vi "eDyno NVH Accel + RPM Simulator.vi"() -> ()   [LabVIEW 2026]
doc: "eDyno NVH simulator for ORDER ANALYSIS - PXIe-4468 AO0 + AO1 in ONE task (the 4468 AO channels share one timing engine, so they cannot run as two separate tasks).\n\nAO0 = accelerometer: PCB 356A15 (one axis) at Sensitivity mV/g, with the same speed profile and Fault Injection as eDyno NVH Accel Simulator.vi.\nAO1 = motor-shaft speed reference, phase-locked to AO0 (same shaft phase, same samples):\n- Pulse Tach OFF (default): analog voltage proportional to rpm, Tach Scale V per 1000 rpm (default 1 V/1000 rpm, so 4500 rpm = 4.5 V).\n- Pulse Tach ON: once-per-rev square wave, 0 / Pulse High V (default 5 V), 50 % duty, rising edge at shaft angle 0 - a keyphasor for SVT tach-to-speed conversion (1 pulse/rev).\n\nAcquire in a separate VI: AO0 -> an accel AI channel (IEPE OFF, same mV/g), AO1 -> a voltage AI channel (IEPE OFF), both in one AI task so they share the sample clock. Analog mode: rpm = V x 1000 / Tach Scale. Orders are referred to the MOTOR shaft (1x = rpm/60 Hz). Fault Frequencies is the answer key at the current speed.\n\nDefaults: run-up 500 -> 4500 rpm over 30 s (Speed Profile / Run-up Enabled), or constant 3000 rpm. Timing: 3-block AO buffer, DAQmx Write paces the loop, the first write auto-starts the task."
uses:
  <vilib>/DAQmx/miscellaneous.llb/DAQmx Fill In Error Info.vi
panel:
  out "Tach Output (V)":dbl[](graph)
  out "Simulated Acceleration (g)":dbl[](graph)
  out "Fault Frequencies (Hz)":T1={"1x Shaft"=50.0, "2x Misalign"=100.0, "BPFO"=178.5, "Torque Ripple"=1200.0, "PWM Carrier"=16000.0}
  out "Shaft Speed (rpm)":dbl=3000.0
  in  "STOP":bool
  in  "Tach Output":T2={"Pulse Tach 1ppr (OFF = analog rpm)"=FALSE, "Tach Scale (V per 1000 rpm)"=1.0, "Pulse High (V)"=5.0}
  in  "Speed Profile":T3={"Run-up Enabled"=FALSE, "Constant Speed (rpm)"=3000.0, "Run-up Start (rpm)"=500.0, "Run-up End (rpm)"=4500.0, "Run-up Duration (s)"=30.0}
  in  "Sim Config":T4={"Sample Rate (Hz)"=51200.0, "Ref Speed (rpm)"=3000.0, "Baseline 1x (g)"=0.02, "Noise Floor (g rms)"=0.01, "BPFO Order"=3.57, "Resonance (Hz)"=3500.0, "Decay (ms)"=0.8, "Pole Pairs"=4.0, "PWM Carrier (Hz)"=16000.0}
  in  "Fault Injection":T5={"Imbalance ON"=FALSE, "Imbalance (g)"=0.5, "Misalignment ON"=FALSE, "Misalignment (g)"=0.2, "Bearing BPFO ON"=FALSE, "Bearing Impact (g)"=2.0, "Motor Ripple ON"=FALSE, "Torque Ripple (g)"=0.3, "PWM Noise ON"=FALSE, "PWM Level (g)"=0.05}
  in  "DAQ Settings":T6={"Device"="PXI2Slot4", "AO Channels (accel+tach)"="ao0:1", "Sample Rate (S/s)"=51200.0, "Samples per Block"=5120, "Sensitivity (mV/g)"=100.0, "AO Range (V)"=10.0}
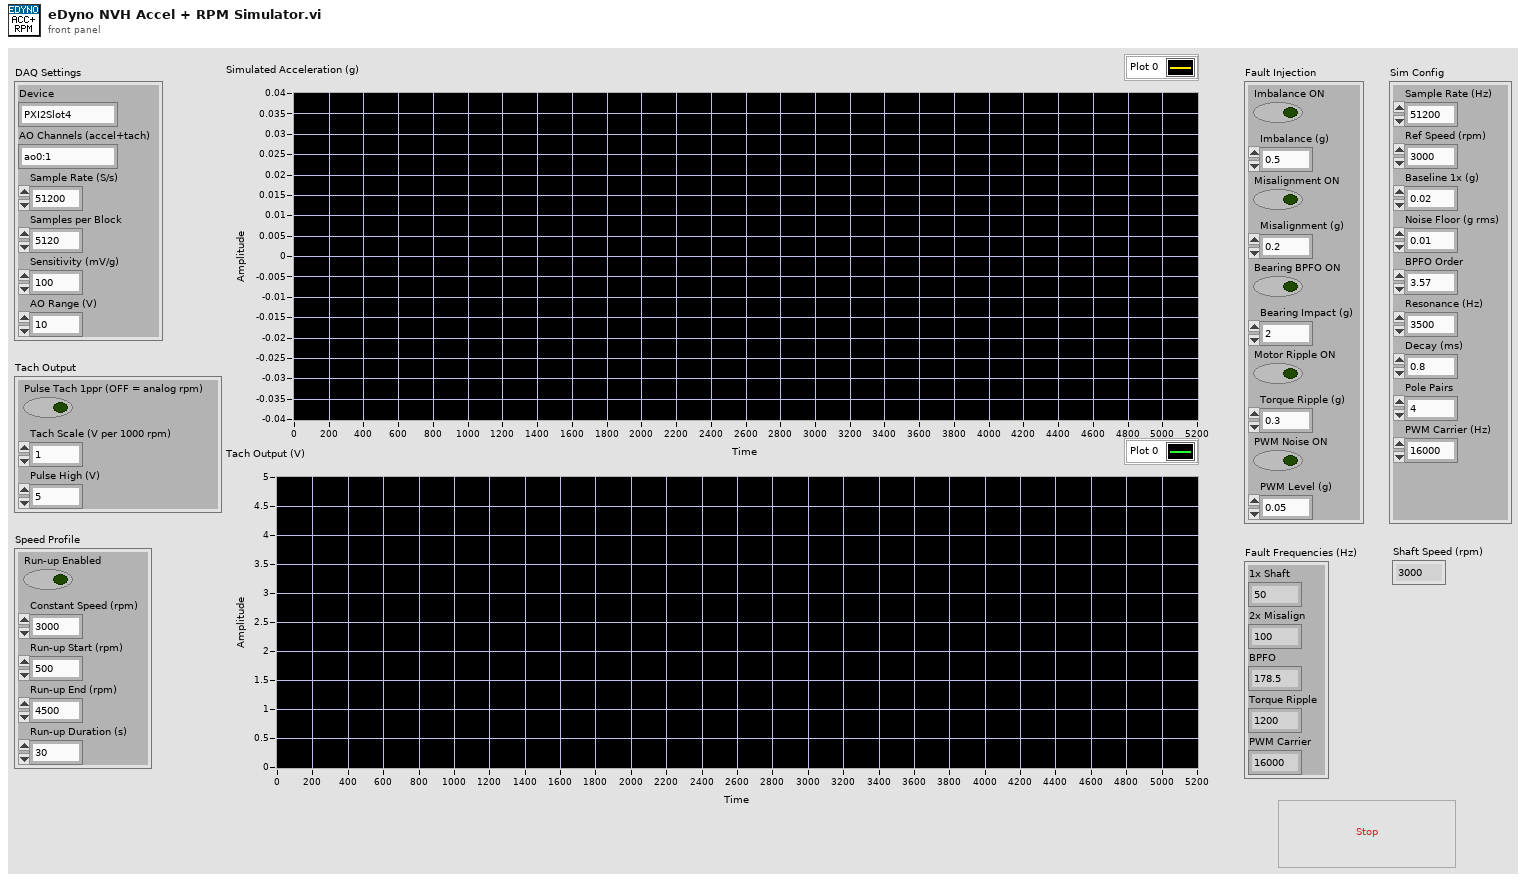
[diagram p1: front panel]
types:
  T1 = cluster{"1x Shaft":dbl, "2x Misalign":dbl, "BPFO":dbl, "Torque Ripple":dbl, "PWM Carrier":dbl}
  T2 = cluster{"Pulse Tach 1ppr (OFF = analog rpm)":bool, "Tach Scale (V per 1000 rpm)":dbl, "Pulse High (V)":dbl}
  T3 = cluster{"Run-up Enabled":bool, "Constant Speed (rpm)":dbl, "Run-up Start (rpm)":dbl, "Run-up End (rpm)":dbl, "Run-up Duration (s)":dbl}
  T4 = cluster{"Sample Rate (Hz)":dbl, "Ref Speed (rpm)":dbl, "Baseline 1x (g)":dbl, "Noise Floor (g rms)":dbl, "BPFO Order":dbl, "Resonance (Hz)":dbl, "Decay (ms)":dbl, "Pole Pairs":dbl, "PWM Carrier (Hz)":dbl}
  T5 = cluster{"Imbalance ON":bool, "Imbalance (g)":dbl, "Misalignment ON":bool, "Misalignment (g)":dbl, "Bearing BPFO ON":bool, "Bearing Impact (g)":dbl, "Motor Ripple ON":bool, "Torque Ripple (g)":dbl, "PWM Noise ON":bool, "PWM Level (g)":dbl}
  T6 = cluster{"Device":string, "AO Channels (accel+tach)":string, "Sample Rate (S/s)":dbl, "Samples per Block":i32, "Sensitivity (mV/g)":dbl, "AO Range (V)":dbl}
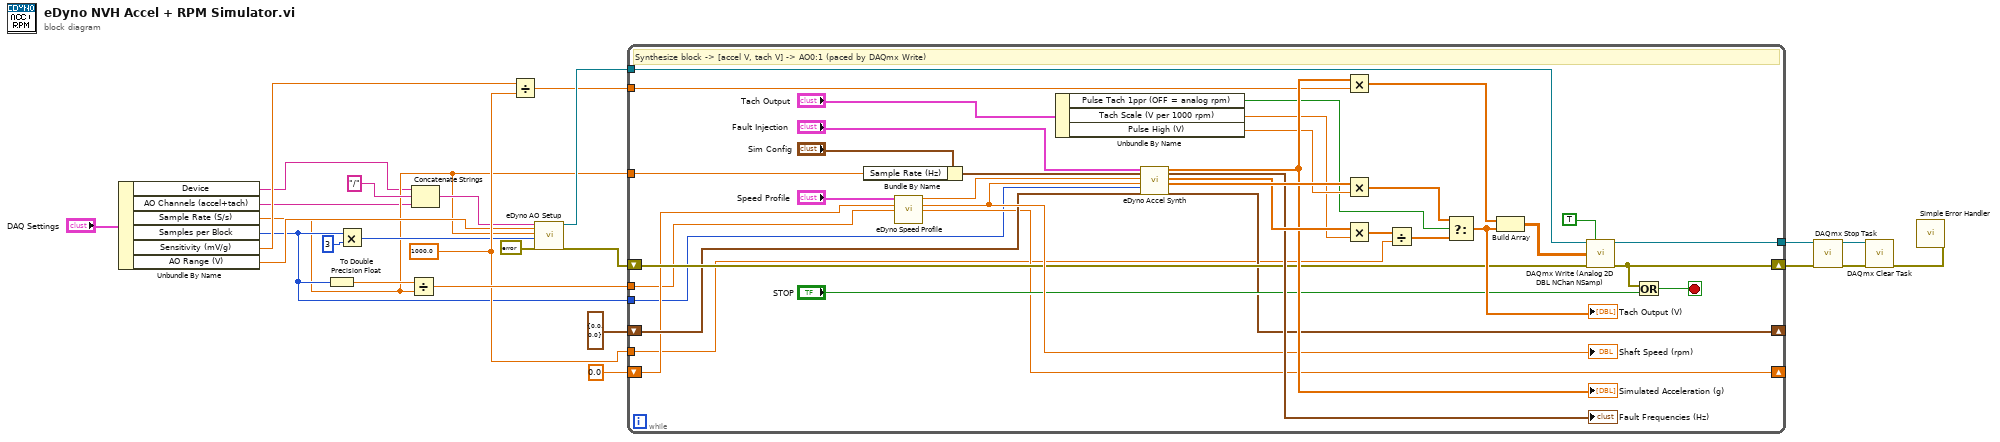
[diagram p0: block diagram]
diagram:
  w13 = 1000.0 ("1000")
  n1 = Unbundle By Name("DAQ Settings") -> ("Device"=w2:string, "AO Channels (accel+tach)"=w3:string, "Sample Rate (S/s)"=w4:dbl, "Samples per Block"=w5:i32, "Sensitivity (mV/g)"=w6:dbl, "AO Range (V)"=w7:dbl)
  n2 = To Double Precision Float(number=w5) -> (double precision float=w15:dbl)
  n3 = Multiply(x=w5, y=3 ("3 blocks")) -> (x*y=w11:i32)
  n4 = Divide(x=w15, y=w4) -> (x/y=w16:dbl)
  n5 = Concatenate Strings(w2, "/" ("slash"), w3) -> (w9:string)
  n6 = Divide(x=w6, y=w13) -> (x/y=w14:dbl)
  n7 = call "eDyno AO Setup.vi"("AO Physical Channel"=w9, "AO Range (V)"=w7, "Sample Rate (S/s)"=w4, "Buffer Samples"=w11, "error in"=errorcluster {"status"=FALSE, "code"=0, "source"=""} ("no error")) -> ("task out"=w17:refnum<k21>, "error out"=w18:errorcluster)  [unwired: 13 in]
  n8 = while {
    tunnel: w13 -> [w31]
    shift-right: [w33] -> _
    shift-left: 0.0 ("run-up t0 (s)") -> [w32]
    shift-right: [w35] -> _
    shift-left: cluster{"Shaft Rev":dbl, "Sample Index":dbl} {"Shaft Rev"=0.0, "Sample Index"=0.0} ("initial synth state") -> [w34]
    tunnel: w4 -> [w27]
    tunnel: w5 -> [w28]
    tunnel: w14 -> [w29]
    tunnel: w17 -> [w26]
    tunnel: w16 -> [w30]
    shift-right: [w37] -> w21
    shift-left: w18 -> [w36]
    tunnel: [w60] -> w22
    stop <- w61 stop-if-true
    # "Synthesize block -> [accel V, tach V] -> AO0:1 (paced by DAQmx Write)"
    n9 = Bundle By Name(cluster="Sim Config", "Sample Rate (Hz)"=w27) -> (w48:T4)
    n10 = call "eDyno Speed Profile.vi"("Speed Profile"="Speed Profile", "t in (s)"=w32, "Block Duration (s)"=w30) -> ("rpm start"=w46:dbl, "rpm end"=w47:dbl, "t out (s)"=w33:dbl)  [unwired: 10 in]
    "Shaft Speed (rpm)" <- w47
    n11 = Unbundle By Name("Tach Output") -> ("Pulse Tach 1ppr (OFF = analog rpm)"=w42:bool, "Tach Scale (V per 1000 rpm)"=w43:dbl, "Pulse High (V)"=w44:dbl)
    n12 = call "eDyno Accel Synth.vi"("Fault Injection"="Fault Injection", "Sim Config"=w48, "rpm start"=w46, "rpm end"=w47, "Samples"=w28, "State in"=w34) -> ("Accel (g)"=w49:dbl[], "Fault Frequencies (Hz)"=→"Fault Frequencies (Hz)":T1, "Speed (rpm)"=w51:dbl[], "Tach Pulse 1ppr (0/1)"=w52:dbl[], "State out"=w35:cluster{"Shaft Rev":dbl, "Sample Index":dbl})  [unwired: 9 in]
    "Simulated Acceleration (g)" <- w49
    n13 = Multiply(x=w49, y=w29) -> (x*y=w53:dbl[])
    n14 = Multiply(x=w52, y=w44) -> (x*y=w56:dbl[])
    n15 = Multiply(x=w51, y=w43) -> (x*y=w54:dbl[])
    n16 = Divide(x=w54, y=w31) -> (x/y=w55:dbl[])
    n17 = Select(t=w56, s=w42, f=w55) -> (s? t:f=w57:dbl[])
    "Tach Output (V)" <- w57
    n18 = Build Array(w53, w57) -> (w58:dbl[][])
    n19 = call <vilib>:"DAQmx Write (Analog 2D DBL NChan NSamp).vi"("task/channels in"=w26, "auto start"=TRUE, "data"=w58, "error in"=w36) -> ("task out"=w60:refnum<k21>, "error out"=w37:errorcluster)  [unwired: 9 in, 1 out]
    n20 = Or(x=w37, y="STOP") -> (x .or. y?=w61:bool)
  }
  n21 = call <vilib>:"DAQmx Stop Task.vi"("task/channels in"=w22, "error in"=w21) -> ("task out"=w23:refnum<k21>, "error out"=w24:errorcluster)  [unwired: 12 in]
  n22 = call <vilib>:"DAQmx Clear Task.vi"("task in"=w23, "error in"=w24) -> ("error out"=w25:errorcluster)  [unwired: 13 in]
  n23 = call <vilib>:"Simple Error Handler.vi"("error in (no error)"=w25) -> ()  [unwired: 4 in, 5 out]
